vi "TestActor.vi"() -> ()   [LabVIEW 2021]
uses:
  Channel.lvlib
panel:
  in  "Config File":path=path "C:/Users/averna/Documents/LV Gym DEMO/Factory Pattern/Channels/Files/Test.ini"
  in  "Plugins Folder":path=path "C:/Users/averna/Documents/LV Gym DEMO/Factory Pattern"
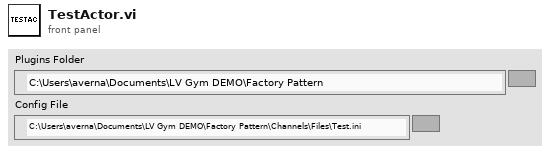
[diagram p1: front panel]
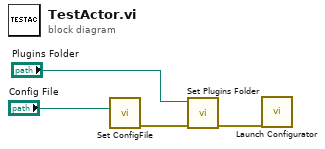
[diagram p0: block diagram]
diagram:
  n1 = call "Set ConfigFile.vi"("Plugins Folder"="Config File") -> ("error out"=w4:errorcluster)  [unwired: 10 in]
  n2 = call "Set Plugins Folder.vi"("error in (no error)"=w4, "Config File"="Plugins Folder") -> ("error out"=w1:errorcluster)  [unwired: 9 in]
  n3 = call "Launch Configurator.vi"("error in (no error)"=w1) -> ()  [unwired: 10 in, 1 out]
